vi "ReadChannels.vi"(8 "error in (no error)":errorcluster, 11 "ChannelsManager in":refnum<class "ChannelsManager.lvclass">) -> (0 "error out":errorcluster, 2 "Channels":refnum<class "Channel.lvclass">[](array[class]), 3 "ChannelsManager out":refnum<class "ChannelsManager.lvclass">)   [LabVIEW 2021, in "Channel.lvlib" / "ChannelsManager.lvlib" / "ChannelsManager.lvclass"]
uses:
  ChannelsManager.lvclass
  Channel_class/Channel.lvclass
  ChannelsManager.lvclass/ChannelsManager.ctl
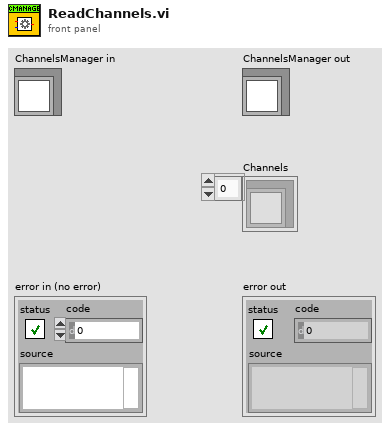
[diagram p1: front panel]
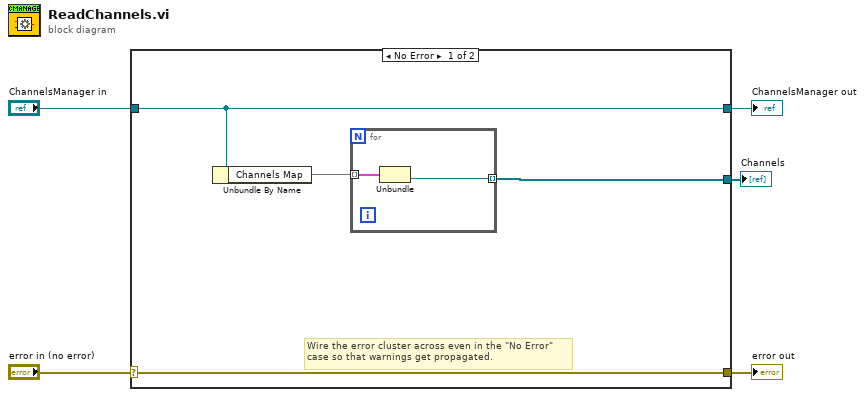
[diagram p0: block diagram]
diagram:
  n1 = case shown="No Error" "error in (no error)" {
    selector: "error in (no error)" -> [w9 w13]
    tunnel: [w9 w13] -> w4
    tunnel: [w8 w12] -> w2
    tunnel: "ChannelsManager in" -> [w8 w12]
    tunnel: [w6 _] -> w1
    frame No Error {
      # "Wire the error cluster across even in the \"No Error\"\ncase so that warnings get propagated."
      n2 = Unbundle By Name(w8) -> ("Channels Map"=w7:map{string, refnum<class "Channel.lvclass">})
      n3 = for {
        tunnel: w7 -> [w11] mode=indexing
        tunnel: [w10] -> w6 mode=indexing
        n4 = Unbundle(w11) -> ("Channel"=w10:refnum<class "Channel.lvclass">)  [unwired: 1 out]
      }
    }
    frame Error {
    }
  }
  "error out" <- w4
  "ChannelsManager out" <- w2
  "Channels" <- w1
